vi "CANsub_Parse_IDs.vi"(8 "error in (no error)":errorcluster, 11 "response":string) -> (0 "error out":errorcluster, 3 "ids":i32[](array[numeric]))   [LabVIEW 2021, in "CANsub_Common.lvlib"]
doc: "Parses a CANsub JSON list of IDs (filters or transmit sequences) into an I32 array. An empty list gives an empty array."
uses:
  CANsub_Common.lvlib
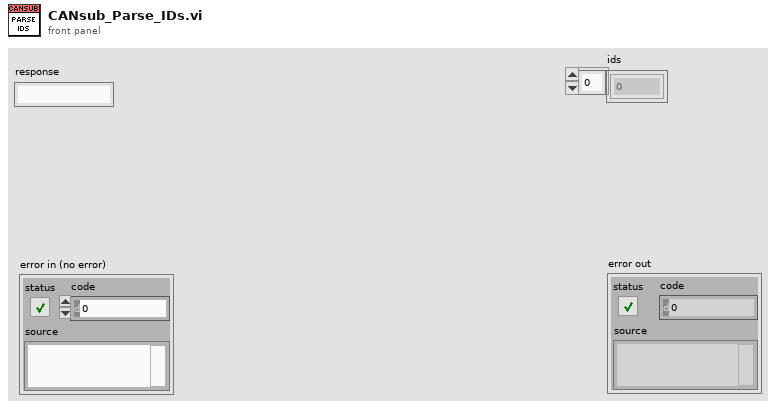
[diagram p1: front panel]
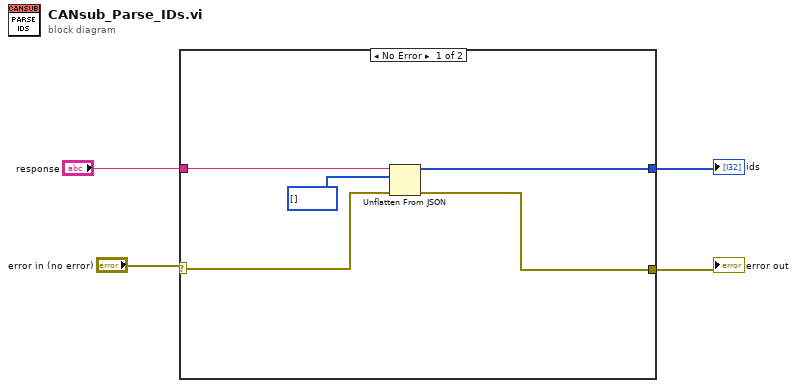
[diagram p0: block diagram]
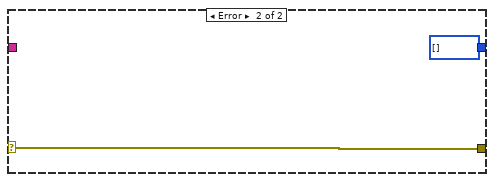
[diagram p2: hidden frame]
diagram:
  n1 = case shown="No Error" "error in (no error)" {
    selector: "error in (no error)" -> [w5 w11]
    tunnel: [w6 w11] -> w4
    tunnel: "response" -> [w9 _]
    tunnel: [w7 i32[] []] -> w1
    frame No Error {
      n2 = Unflatten From JSON(JSON string=w9, type and defaults=i32[] [], error in (no error)=w5) -> (value=w7:i32[], error out=w6:errorcluster)  [unwired: 4 in]
    }
    frame Error {
    }
  }
  "error out" <- w4
  "ids" <- w1
